vi "get SCPI Prefix Command for N9020 Measurement Preset.vi"(8 "error in (no error)":errorcluster, 11 "Keysight 9020A in":refnum<class "Keysight 9020A.lvclass">) -> (0 "error out":errorcluster, 2 "SCPI Prefix Command":string, 3 "Keysight 9020A out":refnum<class "Keysight 9020A.lvclass">)   [LabVIEW 2023, in "Spectrum Analyzer.lvlib" / "Keysight 9020A.lvclass"]
uses:
  Keysight 9020A.lvclass
  Keysight 9020A.lvclass/Keysight 9020A.ctl
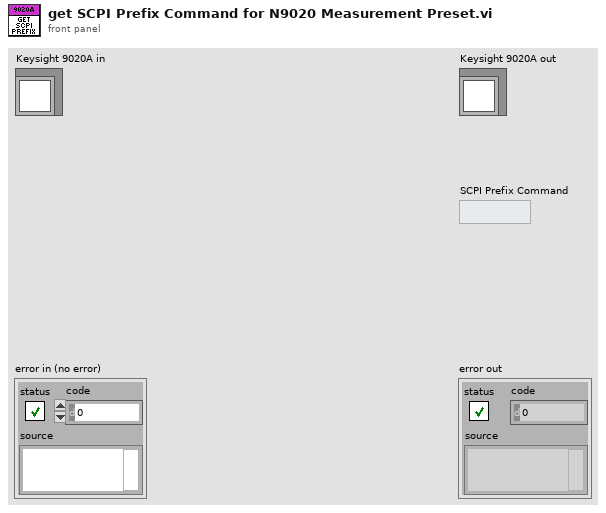
[diagram p1: front panel]
types:
  T1 = typedef "Spectrum Analyzer.lvlib/TYPE Measurement Preset.ctl" = enum16{"Sweep SA Mode", "Channel Power", "Occupied BW", "ACP", "Spurious Emission", "Spurious Emission Mask", "Burst Power (Transmit Power)"}
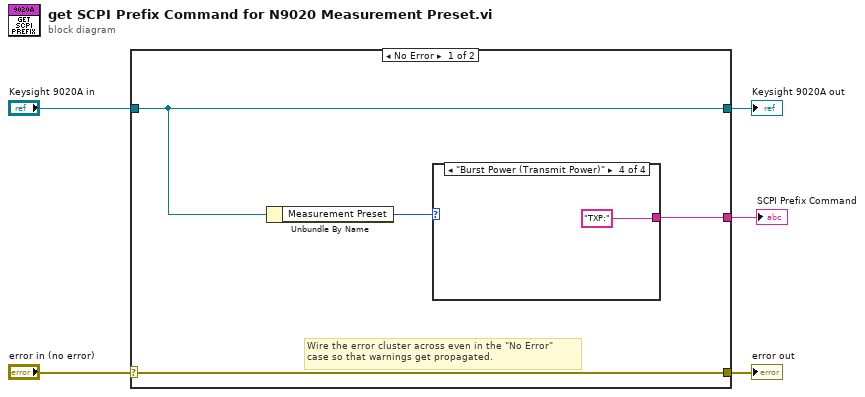
[diagram p0: block diagram]
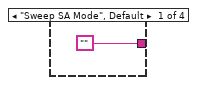
[diagram p2: hidden frame]
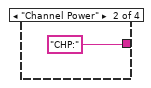
[diagram p3: hidden frame]
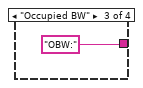
[diagram p4: hidden frame]
diagram:
  n1 = case shown="No Error" "error in (no error)" {
    selector: "error in (no error)" -> [w9 w15]
    tunnel: [w9 w15] -> w4
    tunnel: [w8 w14] -> w2
    tunnel: "Keysight 9020A in" -> [w8 w14]
    tunnel: [w6 _] -> w1
    frame No Error {
      # "Wire the error cluster across even in the \"No Error\"\ncase so that warnings get propagated."
      n2 = Unbundle By Name(w8) -> ("Measurement Preset"=w7:T1)
      n3 = case shown="\"Burst Power (Transmit Power)\"" w7 {
        tunnel: ["" "CHP:" "OBW:" "TXP:"] -> w6
        frame "Sweep SA Mode", Default {
        }
        frame "Channel Power" {
        }
        frame "Occupied BW" {
        }
        frame "Burst Power (Transmit Power)" {
        }
      }
    }
    frame Error {
    }
  }
  "error out" <- w4
  "Keysight 9020A out" <- w2
  "SCPI Prefix Command" <- w1
